vi "Test Lockin Restart Under Load.vi"(8 "error in (no error)":errorcluster) -> (0 "caraya error out":errorcluster)   [LabVIEW 2019]
uses:
  <userlib>/LevyLab/Instrument Framework/Instrument Types/Lockin/Typedefs/LockinAPI.getState.states--enum.ctl
  src/Instrument.Lockin/Instrument.Lockin.lvclass
  <vilib>/addons/_JKI Toolkits/Caraya/classes/Assert/Assert True.vi
  <vilib>/addons/_JKI Toolkits/Caraya/classes/Test/Test.lvclass
  <vilib>/addons/_JKI Toolkits/Caraya/classes/Assert/Assert.lvclass
  <userlib>/LevyLab/Instrument Framework/Instrument Types/Lockin/Instrument.LockinAPI.lvclass
panel:
  out "codes":i32[](array[numeric])
  in  "stop":bool
  out "client error out":errorcluster
  out "state":T1=enum."created"
  out "code":i32
  out "timer":u32
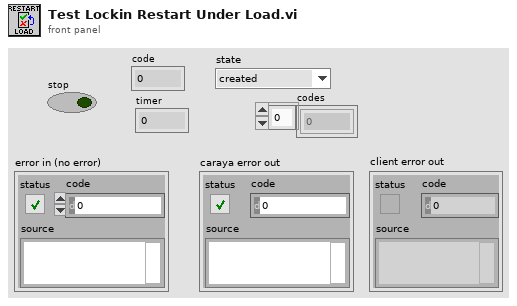
[diagram p1: front panel]
types:
  T1 = typedef "Instrument.LockinAPI.lvclass/LockinAPI.getState.states--enum.ctl" = enum16{"idle", "created", "started", "stopped", "sweeping"}
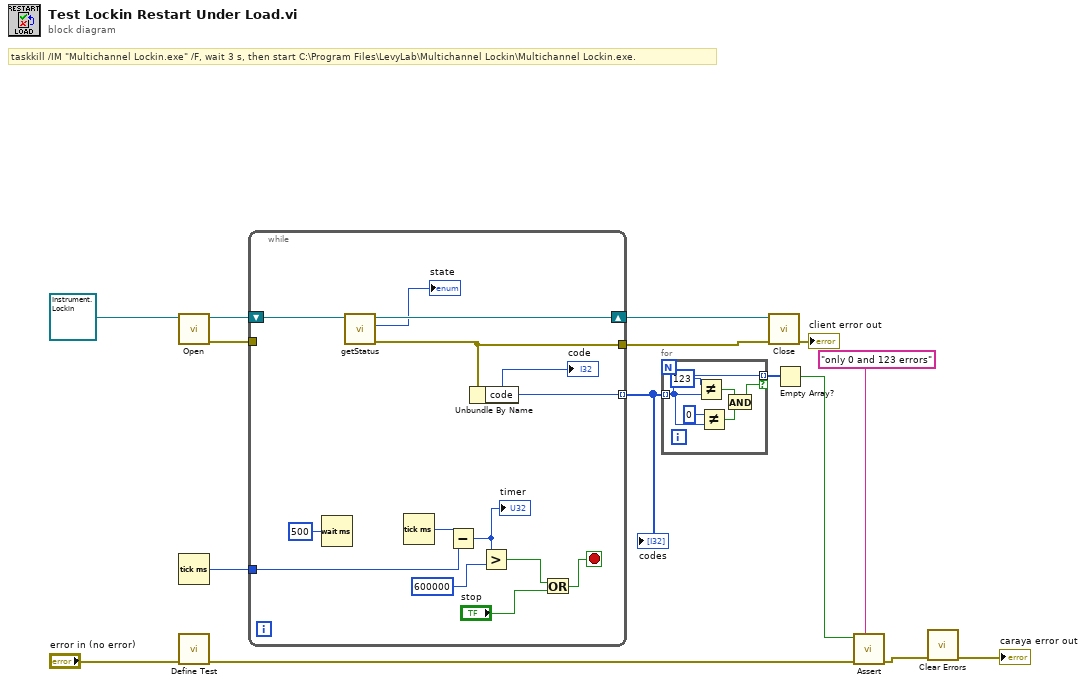
[diagram p0: block diagram]
diagram:
  # "taskkill /IM \"Multichannel Lockin.exe\" /F, wait 3 s, then start C:\\Program Files\\LevyLab\\Multichannel Lockin\\Multichannel Lockin.exe."
  n1 = call-dynamic "Open.vi"("Instrument.Lockin in"=refnum<class "Instrument.Lockin.lvclass"> refnum ("Instrument.Lockin.lvlib:Instrument.Lockin.lvclass")) -> ("error out"=w4:errorcluster, "Instrument.Lockin out"=w5:refnum<class "Instrument.Lockin.lvclass">)  [unwired: 9 in]
  n2 = Tick Count (ms)() -> (millisecond timer value=w13:u32)
  n3 = call <vilib>:"Define Test.vi"("error in (no error)"="error in (no error)") -> ("error out"=w8:errorcluster)  [unwired: 9 in, 1 out]
  n4 = while {
    tunnel: w4 -> [_]
    shift-right: [w21] -> w3
    shift-left: w5 -> [w22]
    tunnel: w13 -> [w27]
    tunnel: [w23] -> w10 mode=indexing
    tunnel: [w20] -> w2
    stop <- w17 stop-if-true
    n5 = Wait (ms)(milliseconds to wait=u32 500) -> ()  [unwired: 1 out]
    n6 = call-dynamic "getStatus.vi"("Instrument.Lockin"=w22) -> ("error out"=w20:errorcluster, "state"=→"state":T1, "Instrument.Lockin"=w21:refnum<class "Instrument.Lockin.lvclass">)  [unwired: 8 in]
    n7 = Tick Count (ms)() -> (millisecond timer value=w28:u32)
    n8 = Subtract(x=w28, y=w27) -> (x-y=w26:u32)
    "timer" <- w26
    n9 = Unbundle By Name(w20) -> ("code"=w23:i32)
    "code" <- w23
    n10 = Greater?(x=w26, y=u32 600000) -> (0:w18:bool)
    n11 = Or(x=w18, y="stop") -> (x .or. y?=w17:bool)
  }
  "codes" <- w10
  n12 = for {
    tunnel: w10 -> [w29] mode=indexing
    tunnel: [w29] -> w7 mode=indexing if=w30
    n13 = Not Equal?(x=123, y=w29) -> (x != y?=w32:bool)
    n14 = Not Equal?(x=0, y=w29) -> (x != y?=w31:bool)
    n15 = And(x=w32, y=w31) -> (x .and. y?=w30:bool)
  }
  n16 = call-dynamic "Close.vi"("error in (no error)"=w2, "Instrument.Lockin in"=w3) -> ("error out"=→"client error out":errorcluster)  [unwired: 8 in, 1 out]
  n17 = Empty Array?(array=w7) -> (empty?=w9:bool)
  n18 = call-poly <vilib>:"Assert.vi"("Label"="only 0 and 123 errors", "error in (no error)"=w8, "True?"=w9) -> ("error out"=w11:errorcluster)  [unwired: 7 in, 1 out]
  n19 = call <vilib>:"Clear Errors.vi"("error in (no error)"=w11) -> ("error out"=→"caraya error out":errorcluster)  [unwired: 5 in, 1 out]
